vi "Prompt File Dialog.vi"(4 "pattern (all files)":string, 6 "pattern label":string, 7 "prompt":string, 8 "error in":errorcluster, 9 "Check if directory (T)":bool=TRUE, 10 "default name":string, 11 "File Path":path) -> (0 "error out":errorcluster, 3 "selected path":path)   [LabVIEW 2017]
doc: "If file path is empty (default) or is <Not A Path> or is a directory, the VI displays a dialog box from which you can select a file. Error 43 occurs if you cancel the dialog box."
uses:
  <vilib>/Utility/sysdir.llb/System Directory Type.ctl
  <vilib>/Utility/error.llb/Error Cluster From Error Code.vi
  <vilib>/ErrorRing/Error Ring.xnode
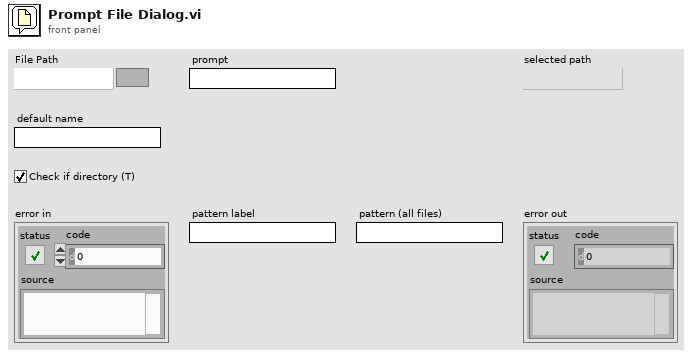
[diagram p1: front panel]
types:
  T1 = typedef "System Directory Type.ctl" = i32
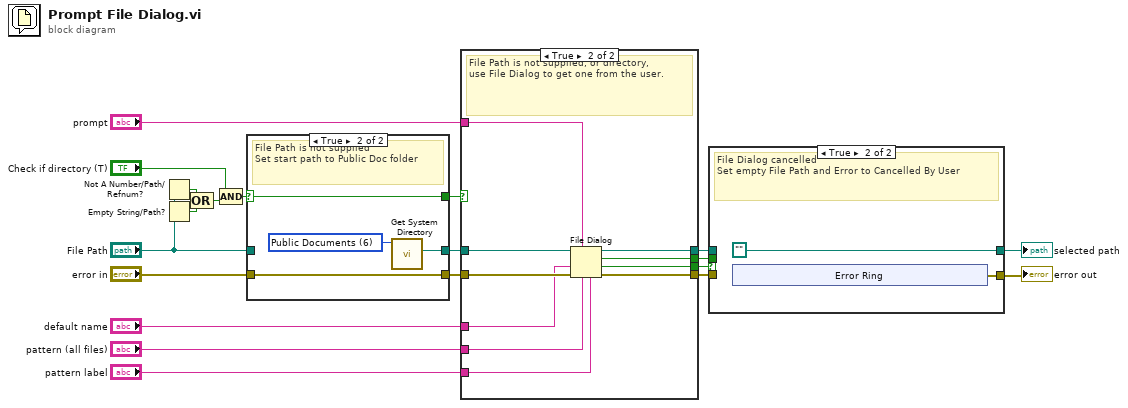
[diagram p0: block diagram]
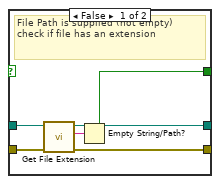
[diagram p2: hidden frame]
diagram:
  n1 = Not A Number/Path/Refnum?(number/path/refnum="File Path") -> (NaN/Path/Refnum?=w17:bool)
  n2 = Empty String/Path?(string/path="File Path") -> (empty?=w16:bool)
  n3 = Compound Arithmetic op=OR(w17, w16) -> (w9:bool)
  n4 = Compound Arithmetic op=AND("Check if directory (T)", w9) -> (w2:bool)
  n5 = case shown="True" w2 {
    selector: w2 -> [_ w29]
    tunnel: "File Path" -> [w26 _]
    tunnel: "error in" -> [w25 w30]
    tunnel: [w23 w30] -> w5
    tunnel: [w24 w27] -> w4
    tunnel: [w21 w29] -> w3
    frame False {
      # "File Path is supplied (not empty) \ncheck if file has an extension"
      n6 = call <vilib>:"Get File Extension.vi"("error in (no error)"=w25, "file"=w26) -> ("error out"=w23:errorcluster, "lowercase file extension"=w22:string, "dup file"=w24:path)  [unwired: 5 in, 2 out]
      n7 = Empty String/Path?(string/path=w22) -> (empty?=w21:bool)
    }
    frame True {
      w28 = T1 6 items=["User Home"=0, "User Desktop"=1, "User Documents"=2, "User Application Data"=3, "User Preferences"=4, "User Temporary"=5, "Public Documents"=6, "Public Application Data"=7, "Public Preferences"=8, "Public Cache"=13, "System Core Libraries"=9, "System Installed Libraries"=10, "Application Files"=11, "Boot Volume Root"=12] ("system directory type")
      # "File Path is not supplied\nSet start path to Public Doc folder"
      n8 = call <vilib>:"Get System Directory.vi"("system directory type"=w28) -> ("system directory"=w27:path)  [unwired: 10 in]
    }
  }
  n9 = case shown="True" w3 {
    tunnel: w5 -> [w31 w42]
    tunnel: [w31 w41] -> w13
    tunnel: "pattern (all files)" -> [_ w40]
    tunnel: "pattern label" -> [_ w39]
    tunnel: "default name" -> [_ w38]
    tunnel: [w32 w37] -> w14
    tunnel: w4 -> [w32 w36]
    tunnel: "prompt" -> [_ w35]
    tunnel: [_ w34] -> w10
    tunnel: [_ w33] -> w15
    frame False {
      # "File Path is supplied (not empty and not a directory)"
    }
    frame True {
      # "File Path is not supplied, or directory,\nuse File Dialog to get one from the user."
      n10 = File Dialog(4:w39, 6:w40, 7:w35, 8:w42, 9:w38, 11:w36) -> (0:w41:errorcluster, 1:w33:bool, 2:w34:bool, 3:w37:path)  [unwired: 1 in]
    }
  }
  n11 = case shown="True" w15 {
    tunnel: w14 -> [w44 _]
    tunnel: w13 -> [w43 _]
    tunnel: [w44 path ""] -> w12
    tunnel: [w43 w45] -> w11
    tunnel: w10 -> [_ _]
    frame False {
      # "File path supplied or selected"
    }
    frame True {
      # "File Dialog cancelled\nSet empty File Path and Error to Cancelled By User"
      n12 = xnode "Error Ring"() -> ("error out"=w45:errorcluster)
    }
  }
  "error out" <- w11
  "selected path" <- w12
